vi "Toolbar Manage Button Click Event.vi"(6 "Index In":i32, 7 "Button":T1(ring), 8 "error in (no Error)":errorcluster, 9 "Button Index":i32, 10 "Button States In":refnum<class "Button.lvclass">[](array[class]), 11 "Data In":T2) -> (0 "error out":errorcluster, 1 "Data Changed ?":bool, 2 "Button States Out":refnum<class "Button.lvclass">[](array[class]), 3 "Data Out":T2, 4 "Index Out":i32)   [LabVIEW 2012, in "Toolbar.xctl"]
doc: "Process Left Button Clicks on the toolbar taking account of the button state and type."
uses:
  Toolbar.xctl
  Button_Class/Button.lvclass
  Toolbar Data.ctl
  Button_Class/Type Defs/Button Events.ctl
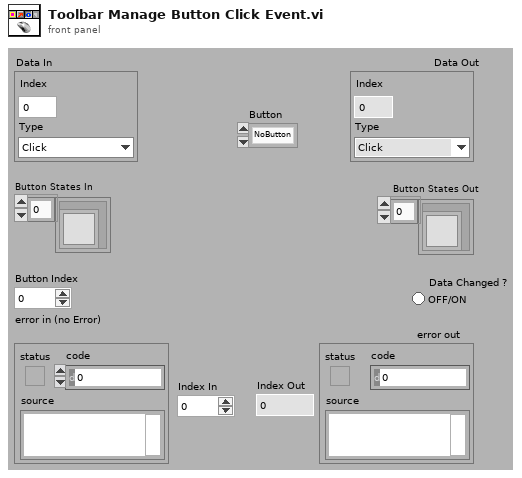
[diagram p1: front panel]
types:
  T1 = enum16{"NoButton", "Left Button", "Right Button", "Middle Button"}
  T2 = typedef "Toolbar.xctl/Toolbar Data.ctl" = cluster{"Index":i32, "Type":T3}
  T3 = typedef "Button.lvclass/Button Events.ctl" = enum16{"Click", "Latch", "Unlatch"}
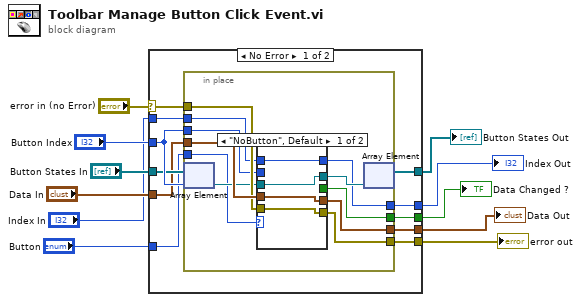
[diagram p0: block diagram]
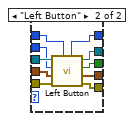
[diagram p2: hidden frame]
diagram:
  n1 = case shown="No Error" "error in (no Error)" {
    selector: "error in (no Error)" -> [w17 w50]
    tunnel: [w22 _] -> w11
    tunnel: [w21 _] -> w10
    tunnel: "Button Index" -> [w20 _]
    tunnel: "Button States In" -> [w19 _]
    tunnel: [w18 w49] -> w7
    tunnel: [w16 w50] -> w5
    tunnel: "Data In" -> [w15 w49]
    tunnel: [w14 w48] -> w3
    tunnel: "Index In" -> [w13 w48]
    tunnel: "Button" -> [w12 _]
    frame No Error {
      n2 = in-place {
        in-place-border: w20 -> [w26]
        in-place-border: w15 -> [w33]
        in-place-border: [w32] -> w16
        in-place-border: w17 -> [w31]
        in-place-border: [w30] -> w22
        in-place-border: [w29] -> w18
        in-place-border: [w25] -> w14
        in-place-border: w13 -> [w24]
        in-place-border: w12 -> [w23]
        n3 = in-place-array #1(w19, w20) -> (w28:refnum<class "Button.lvclass">)
        n4 = case shown="\"NoButton\", Default" w23 {
          tunnel: w33 -> [w36 w47]
          tunnel: [w35 w46] -> w32
          tunnel: w31 -> [w35 w45]
          tunnel: [_ w44] -> w30
          tunnel: [w36 w43] -> w29
          tunnel: w28 -> [w37 w42]
          tunnel: [w37 w41] -> w27
          tunnel: w26 -> [_ w40]
          tunnel: [w34 w39] -> w25
          tunnel: w24 -> [w34 w38]
          frame "NoButton", Default {
          }
          frame "Left Button" {
            n5 = call-dynamic "Left Button.vi"("Index In in"=w38, "error in (no error)"=w45, "Data In"=w47, "Button Index"=w40, "Button in"=w42) -> ("error out"=w46:errorcluster, "Data out"=w43:T2, "Data Changed ?"=w44:bool, "Button out"=w41:refnum<class "Button.lvclass">, "Index In out"=w39:i32)  [unwired: 2 in]
          }
        }
        n6 = in-place-array #1(w27) -> (w21:refnum<class "Button.lvclass">[])  [unwired: 1 out]
      }
    }
    frame Error {
    }
  }
  "Data Changed ?" <- w11
  "Button States Out" <- w10
  "Data Out" <- w7
  "error out" <- w5
  "Index Out" <- w3
